vi "Task Loop.vi"(8 "error in (no error)":errorcluster, 11 "SimTask in":refnum<class "SimTask.lvclass">) -> (0 "error out":errorcluster)   [LabVIEW 2020, in "VolatusDemo.lvlib" / "SimTask.lvclass"]
uses:
  SimTask.lvclass
  lv-vecto/Vecto/Group/Group.lvclass
  Volatus/Task/Task.lvclass
  VolatusData/DataHandlerAPI/DataHandlerAPI.lvclass
  C:/dev/lv20CE/relink/lv-volatus/Volatus/Task/Task.lvclass
panel:
  in  "E":dbl(slide) scale=0.0..100.0
  in  "D":dbl(slide) scale=0.0..100.0
  in  "C":dbl(slide) scale=0.0..100.0
  in  "B":dbl(slide) scale=0.0..100.0
  in  "A":dbl(slide) scale=0.0..100.0
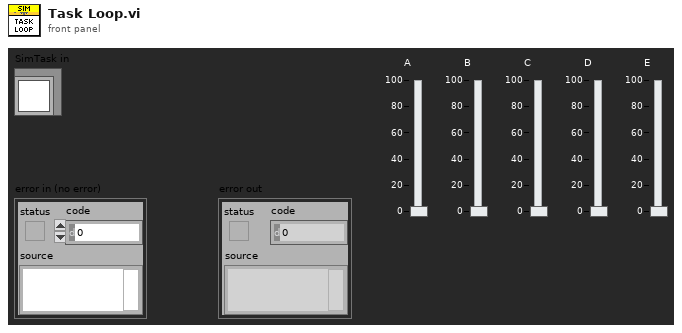
[diagram p1: front panel]
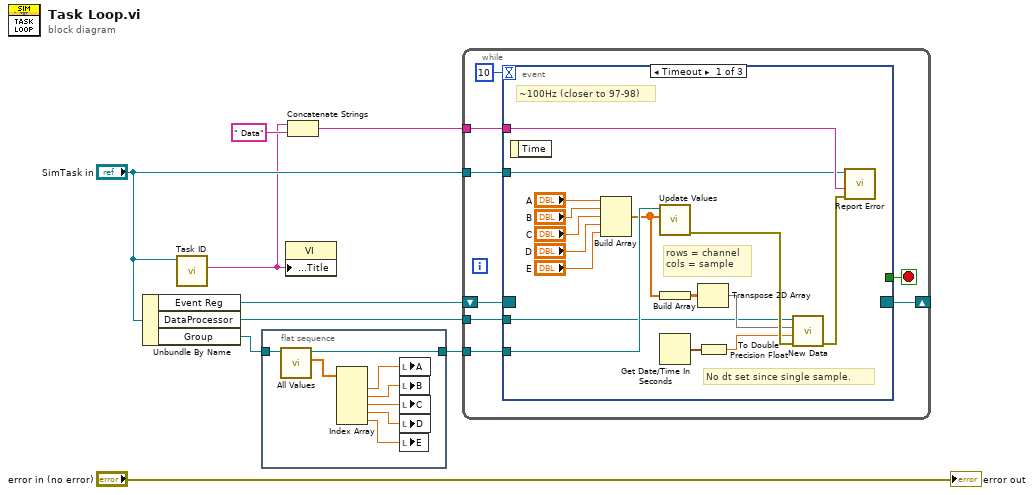
[diagram p0: block diagram]
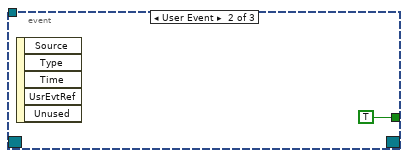
[diagram p2: hidden frame]
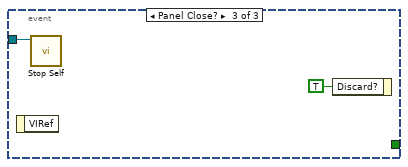
[diagram p3: hidden frame]
diagram:
  n1 = Unbundle By Name("SimTask in") -> ("Event Reg"=w8:refnum<event-registration>, "DataProcessor"=w1:refnum<class "DataHandlerAPI.lvclass">, "Group"=w2:refnum<class "Group.lvclass">)
  n2 = call-dynamic "Task ID.vi"("Task in"="SimTask in") -> ("Task ID"=w4:string)  [unwired: 8 in, 2 out]
  n3 = flat-sequence {
    tunnel: [w16] -> w3
    tunnel: w2 -> [w17]
    frame #0 {
      n4 = call "All Values.vi"("Group in"=w17) -> ("Scaled"=w15:dbl[], "Group out"=w16:refnum<class "Group.lvclass">)  [unwired: 6 in, 3 out]
      n5 = Index Array(array=w15) -> (element #1=w12:dbl, element #2=w13:dbl, element #3=w14:dbl, element #4=w11:dbl, element #5=w10:dbl)  [unwired: 5 in]
      n6 = local write "A"(w12) -> ()
      n7 = local write "B"(w13) -> ()
      n8 = local write "C"(w14) -> ()
      n9 = local write "D"(w11) -> ()
      n10 = local write "E"(w10) -> ()
    }
  }
  n11 = property class="VI"("Front Panel.Title"=w4) -> ()  [unwired: 2 in, 2 out]
  n12 = Concatenate Strings(w4, " Data" ("string")) -> (w6:string)
  n13 = while {
    shift-right: [w24] -> _
    shift-left: w8 -> [w25]
    tunnel: "SimTask in" -> [w21]
    tunnel: w3 -> [w20]
    tunnel: w6 -> [w19]
    tunnel: w1 -> [w18]
    stop <- w23 stop-if-true
    n14 = event shown="[0] Timeout" {
      selector: w25 -> [_ _ _]
      dyn-events: [_ _ _] -> w24
      timeout: 10 -> [_ _ _]
      tunnel: [_ TRUE _] -> w23
      tunnel: w21 -> [w26 _ w43]
      tunnel: w20 -> [w35 _ _]
      tunnel: w19 -> [w28 _ _]
      tunnel: w18 -> [w27 _ _]
      event Timeout {
        # "No dt set since single sample."
        # "~100Hz (closer to 97-98)"
        # "rows = channel\ncols = sample"
        n15 = event-data() -> ()  [unwired: 1 in, 1 out]
        n16 = Build Array("A", "B", "C", "D", "E") -> (w34:dbl[])
        n17 = call "Update Values.vi"("Values"=w34, "Group in"=w35) -> ("error out"=w41:errorcluster)  [unwired: 8 in, 1 out]
        n18 = Build Array(w34) -> (w33:dbl[][])
        n19 = Get Date/Time In Seconds() -> (seconds since 1Jan1904=w32:timestamp)
        n20 = Transpose 2D Array(2D array=w33) -> (transposed array=w29:dbl[][])
        n21 = To Double Precision Float(number=w32) -> (double precision float=w31:dbl)
        n22 = call "New Data.vi"("error in (no error)"=w41, "t0"=w31, "Data"=w29, "DataHandlerAPI in"=w27) -> ("error out"=w30:errorcluster)  [unwired: 6 in, 1 out]
        n23 = call "Report Error.vi"("error in (no error)"=w30, "Message"=w28, "Task in"=w26) -> ()  [unwired: 7 in, 2 out]
      }
      event User Event {
        n24 = event-data() -> ()  [unwired: 1 in, 5 out]
      }
      event Panel Close? {
        n25 = event-data() -> ()  [unwired: 1 in, 1 out]
        n26 = call "Stop Self.vi"("Task in"=w43) -> ()  [unwired: 9 in, 2 out]
        n27 = event-data("Discard?"=TRUE) -> ()  [unwired: 1 in, 1 out]
      }
    }
  }
  "error out" <- "error in (no error)"
